vi "DAQ Performance Test.vi"() -> ()   [LabVIEW 2021]
uses:
  ChannelCommon/typedef/Benchmark Stats.ctl
  ChannelCommon/typedef/Direction.ctl
  CIF_Iceoryx_Fifo_DAQ.lvclass
  D:/dev/Packages/CIF_Channels_Core/src/CIFChannels/CIFChannels.lvclass
  Iceorxy Utilities/Typedef/DAQ FIFO Config.ctl
  ChannelCommon/typedef/Datatype Waveform.ctl
  <vilib>/Platform/TimedLoop/XDataNode/timing_clust.ctl
  <vilib>/Platform/TimedLoop/XDataNode/nitl_modes.ctl
  <vilib>/Platform/TimedLoop/XDataNode/wakeup.ctl
  ChannelCommon/typedef/TimeStamps.ctl
  CIFChannels/CIFChannels.lvclass/CIFChannels.ctl
  <vilib>/CIF Foundation/CIF Utilities/Statistics/I64/Stats_I64_CIF_U.lvclass/Stats_I64_CIF_U.ctl
  <vilib>/CIF Foundation/CIF Utilities/Statistics/I64/Get Stats.vi
  <vilib>/Platform/TimedLoop/XDataNode/XDataNode.xnode
  <vilib>/Platform/TimedLoop/XDataNode/XDNodeRunTimeDep.lvlib
  ChannelCommon/ChannelCommon.lvlib
  CIFChannels/CIFChannels.lvclass
  Iceorxy Utilities/Iceoryx Channel Utilities.lvlib
panel:
  out "timed out? 2":bool
  out "Channel W (us)":T1
  out "Flatten (us)":T1
  in  "stop":bool
  out "Unflatten (us)":T1
  out "Channel R (us)":T1
  out "timed out?":bool
  out "avg channel":dbl
  out "max channel":dbl
  out "pass":bool
  out "error out":errorcluster
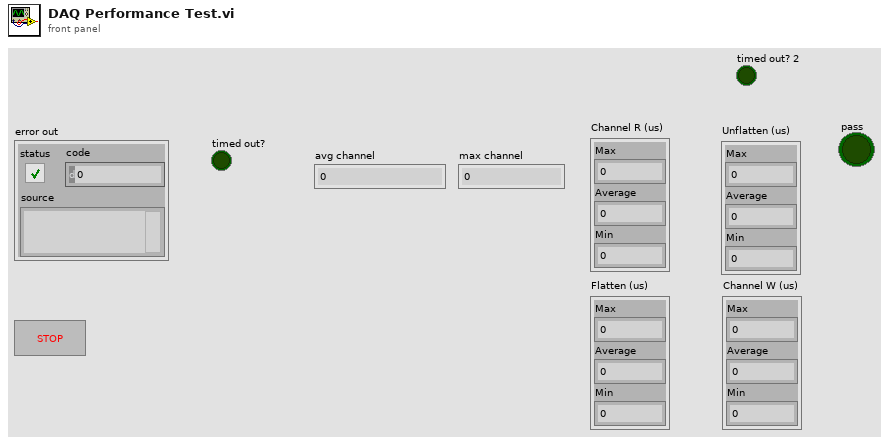
[diagram p1: front panel]
types:
  T1 = typedef "ChannelCommon.lvlib/Benchmark Stats.ctl" = cluster{"Max":i64, "Average":dbl, "Min":i64}
  T2 = typedef "Iceoryx Channel Utilities.lvlib/DAQ FIFO Config.ctl" = cluster{"Max Samples":u64, "Max Channels":u64, "FIFO Flags":cluster{"Backpressure":bool}, "Best Effort Subscribers":u32, "Backpressure Subscribers":u32}
  T3 = typedef "ChannelCommon.lvlib/Direction.ctl" = enum8{"Publisher", "Subscriber"}
  T4 = typedef "ChannelCommon.lvlib/Datatype Waveform.ctl" = cluster{"Measurement":dbl[], "dT":dbl, "Timestamp":i64}
  T5 = typedef "ChannelCommon.lvlib/TimeStamps.ctl" = cluster{"ClockID":u8, "T0":i64, "T_Out":i64}
  T6 = typedef "XDNodeRunTimeDep.lvlib/timing_clust.ctl" = cluster{"Expected End [f-1]":u64, "Actual End [f-1]":u64, "Finished Late? [f-1]":bool, "Expected End [i-1]":u64, "Actual End [i-1]":u64, "Finished Late? [i-1]":bool, "Expected Start [i]":u64, "Actual Start [i]":u64, "Expected Start [f]":u64, "Actual Start [f]":u64, "Source Name":string, "Structure Name":string, "Period":i64, "Deadline":i64, "Offset":i64, "Start":i64, "Priority":i32, "Timeout":i32, "Mode":T7, "Wakeup Reason":T8, "Error":errorcluster, "Source Type":string, "Secondary Source Type":string, "Global End Time":u64, "Global Start Time":u64, "Frame Duration":u64, "Iteration Duration":u64, "Assigned CPU":i32, "I/O Scan Engine Mode":u32}
  T7 = typedef "XDNodeRunTimeDep.lvlib/nitl_modes.ctl" = enum32{"No Change", "Process missed periods, maintain original phase", "Discard missed periods, maintain original phase", "Process missed periods, ignore original phase", "Discard missed periods, ignore original phase"}
  T8 = typedef "XDNodeRunTimeDep.lvlib/wakeup.ctl" = enum32{"Normal", "Aborted", "Asynchronous wakeup", "Timing source error", "Timed loop error", "Timeout"}
  T9 = typedef "ChannelCommon.lvlib/New FIFO Instance Response.ctl" = cluster{"Publisher":string, "Custom Data":u8[]}
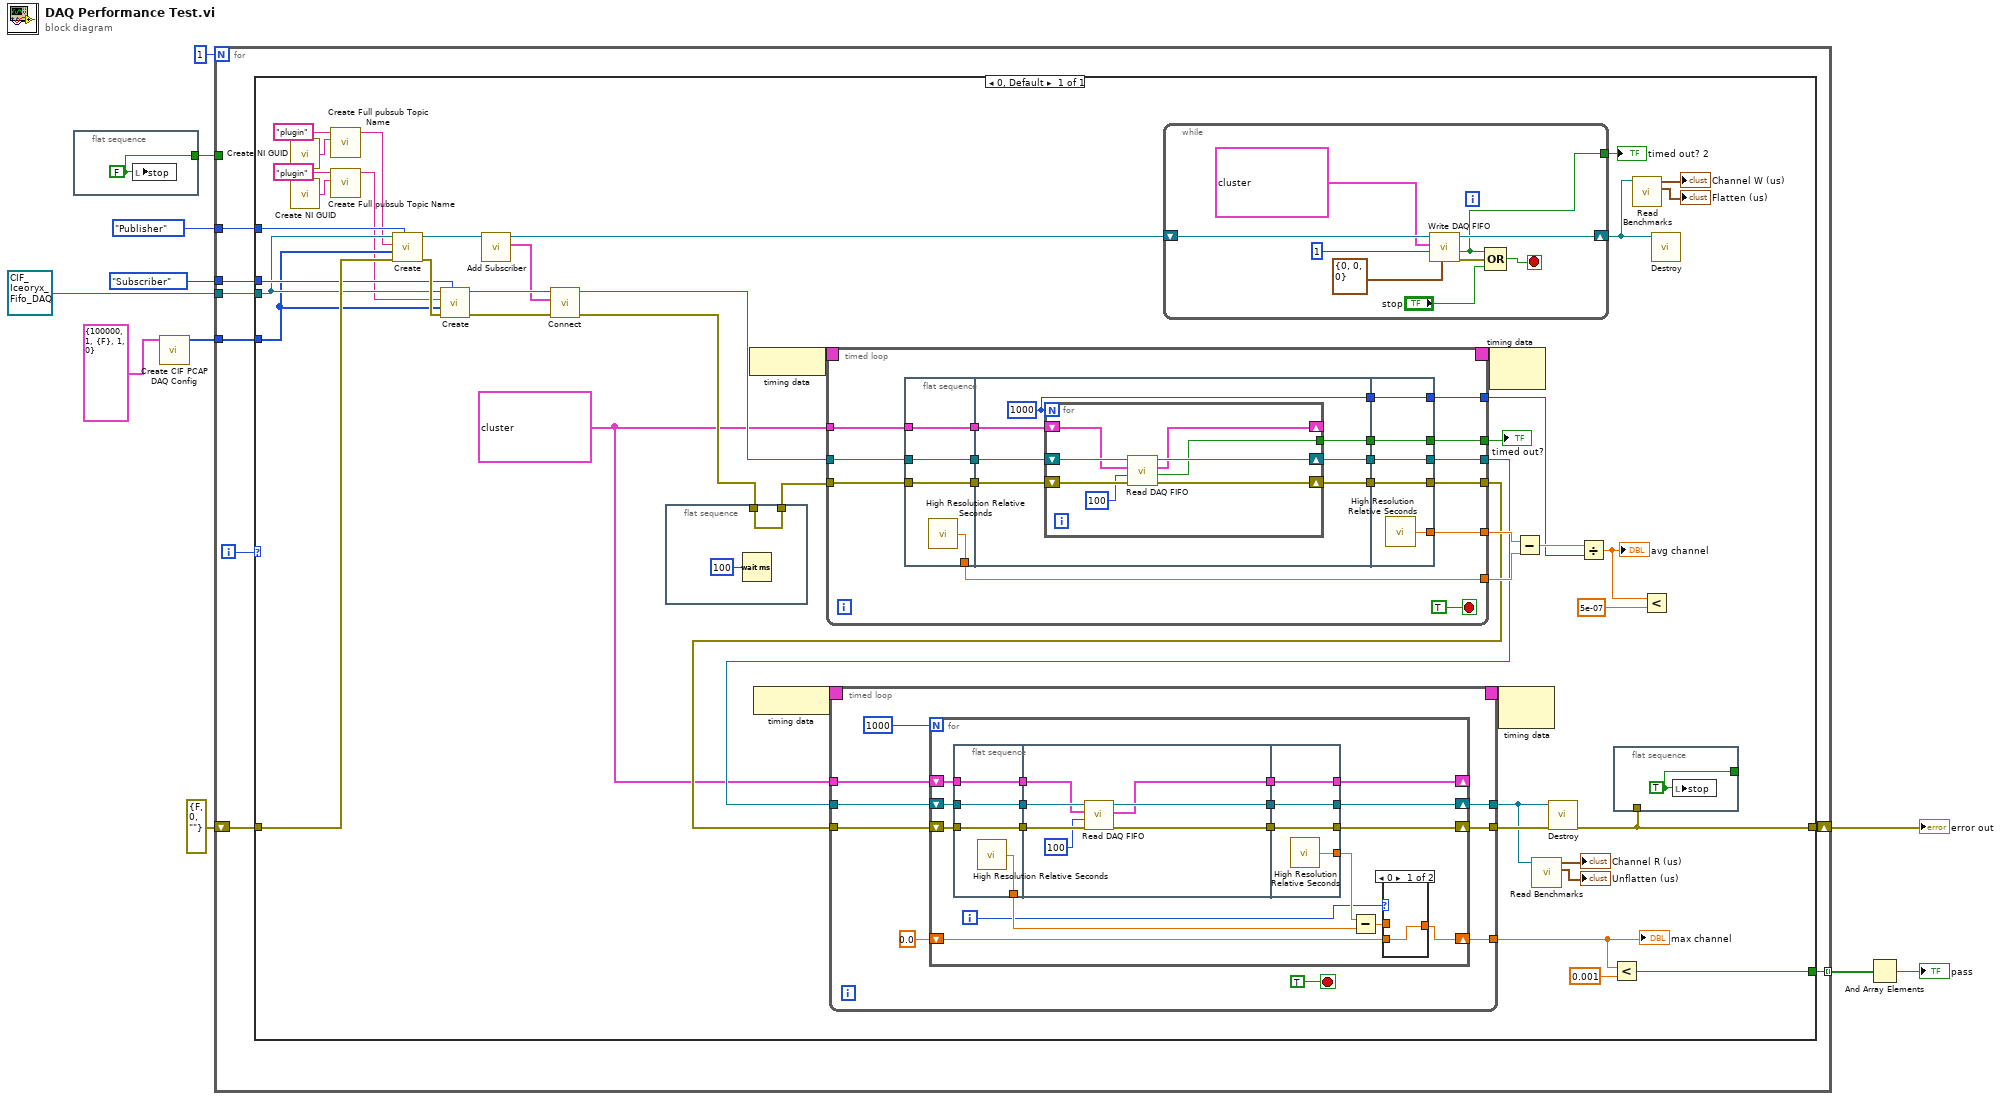
[diagram p0: block diagram]
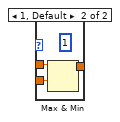
[diagram p2: hidden frame]
diagram:
  n1 = flat-sequence {
    tunnel: [w12] -> w3
    frame #0 {
      w12 = FALSE ("stop")
      n2 = local write "stop"(w12) -> ()
    }
  }
  n3 = call "Create CIF PCAP DAQ Config.vi"("DAQ FIFO Config"=T2 {"Max Samples"=100000, "Max Channels"=1, "FIFO Flags"={"Backpressure"=FALSE}, "Best Effort Subscribers"=1, "Backpressure Subscribers"=0}) -> ("Flattened FIFO Config"=w1:u8[])  [unwired: 10 in]
  n4 = for {
    N: 1 -> [_]
    tunnel: [w20] -> w9 mode=indexing
    shift-right: [w19] -> w11
    shift-left: errorcluster {"status"=FALSE, "code"=0, "source"=""} ("error out") -> [w17]
    tunnel: Direction."Publisher" ("Direction") -> [w16]
    tunnel: Direction."Subscriber" ("Direction") -> [w15]
    tunnel: refnum<class "CIF_Iceoryx_Fifo_DAQ.lvclass"> refnum ("CIF_CIPC_Fifo_U8.lvclass") -> [w14]
    tunnel: w1 -> [w13]
    tunnel: w3 -> [_]
    i -> [w18]
    n5 = case shown="0, Default" w18 {
      tunnel: [w52] -> w20
      tunnel: [w35] -> w19
      tunnel: w17 -> [w50]
      tunnel: w16 -> [w49]
      tunnel: w15 -> [w48]
      tunnel: w14 -> [w47]
      tunnel: w13 -> [w44]
      frame 0, Default {
        w28 = T4[] [{"Measurement"=array[100000 elements], "dT"=3.0, "Timestamp"=121}] ("Data In")
        n6 = call <vilib>:"Create NI GUID.vi"() -> ("NI GUID"=w30:string)
        n7 = call <vilib>:"Create NI GUID.vi"() -> ("NI GUID"=w31:string)
        n8 = call "Create Full pubsub Topic Name.vi"("Topic"=w30, "Plugin name"="plugin") -> ("Full Topic"=w27:string)  [unwired: 8 in, 1 out]
        n9 = call "Create Full pubsub Topic Name.vi"("Topic"=w31, "Plugin name"="plugin") -> ("Full Topic"=w26:string)  [unwired: 8 in, 1 out]
        n10 = call-dynamic "Create.vi"("Direction"=w49, "error in (no error)"=w50, "Custom Config Data"=w44, "Name"=w27, "CIFFIFO in"=w47) -> ("error out"=w51:errorcluster, "CIFFIFO out"=w34:refnum<class "CIF_Iceoryx_Fifo_DAQ.lvclass">)  [unwired: 5 in]
        n11 = call-dynamic "Create.vi"("Direction"=w48, "error in (no error)"=w51, "Custom Config Data"=w44, "Name"=w26, "CIFFIFO in"=w47) -> ("error out"=w45:errorcluster, "CIFFIFO out"=w46:refnum<class "CIF_Iceoryx_Fifo_DAQ.lvclass">)  [unwired: 5 in]
        n12 = call-dynamic "Add Subscriber.vi"("CIF_CIPC_Chn in"=w34) -> ("New FIFO Instance"=w33:T9, "CIF_CIPC_Chn out"=w23:refnum<class "CIF_Iceoryx_Fifo_DAQ.lvclass">)  [unwired: 8 in, 1 out]
        n13 = call-dynamic "Connect.vi"("error in (no error)"=w45, "Connection"=w33, "CIF_Iceoryx_PCAP"=w46) -> ("error out"=w41:errorcluster, "CIF_Iceoryx_PCAP"=w43:refnum<class "CIF_Iceoryx_Fifo_DAQ.lvclass">)  [unwired: 7 in]
        n14 = flat-sequence {
          tunnel: w41 -> [w69]
          tunnel: [w69] -> w40
          frame #0 {
            n15 = Wait (ms)(milliseconds to wait=u32 100) -> ()  [unwired: 1 out]
          }
        }
        n16 = node-c288() -> (w66:T6)
        n17 = node-c288() -> (w64:T6)
        n18 = timed-loop {
          timing: w66 -> [_]
          timing-out: [_] -> w65
          tunnel: w43 -> [w145]
          tunnel: w40 -> [w144]
          tunnel: [w140] -> w58
          tunnel: [w138] -> w57
          tunnel: [w136] -> w62
          tunnel: [w135] -> w61
          tunnel: [w134] -> w59
          tunnel: [w132] -> w39
          tunnel: w28 -> [w129]
          stop <- TRUE stop-if-true
          n19 = flat-sequence {
            tunnel: w144 -> [w148]
            tunnel: w145 -> [w149]
            tunnel: [w149] -> w142
            tunnel: [w148] -> w141
            tunnel: [w147] -> w135
            tunnel: [w146] -> w130
            tunnel: w129 -> [w146]
            tunnel: w142 -> [w156]
            tunnel: w141 -> [w155]
            tunnel: [w154] -> w139
            tunnel: [w153] -> w137
            tunnel: [w152] -> w133
            tunnel: [w151] -> w131
            tunnel: w130 -> [w150]
            tunnel: [w169] -> w140
            tunnel: w139 -> [w169]
            tunnel: [w168] -> w138
            tunnel: w137 -> [w168]
            tunnel: [w167] -> w136
            tunnel: [w166] -> w134
            tunnel: w133 -> [w166]
            tunnel: [w165] -> w132
            tunnel: w131 -> [w165]
            frame #0 {
              n20 = call <vilib>:"High Resolution Relative Seconds.vi"() -> ("relative seconds"=w147:dbl)
            }
            frame #1 {
              w152 = 1000
              n21 = for {
                N: w152 -> [_]
                shift-right: [w161] -> w154
                shift-left: w156 -> [w164]
                shift-right: [w162] -> w153
                shift-left: w155 -> [w163]
                tunnel: [w159] -> w151
                shift-right: [w157] -> _
                shift-left: w150 -> [w158]
                n22 = call-dynamic "Read DAQ FIFO.vi"("error in (no error)"=w163, "Timeout (ms)"=100, "Data In"=w158, "CIFFIFO in"=w164) -> ("error out"=w162:errorcluster, "timed out?"=w159:bool, "Data Out"=w157:T4[], "CIFFIFO out"=w161:refnum<class "CIF_Iceoryx_Fifo_DAQ.lvclass">)  [unwired: 3 in, 1 out]
              }
            }
            frame #2 {
              n23 = call <vilib>:"High Resolution Relative Seconds.vi"() -> ("relative seconds"=w167:dbl)
            }
          }
        }
        "timed out?" <- w39
        n24 = timed-loop {
          timing: w64 -> [_]
          timing-out: [_] -> w63
          tunnel: w58 -> [w87]
          tunnel: w57 -> [w86]
          tunnel: [w84] -> w38
          tunnel: [w83] -> w42
          tunnel: [w80] -> w54
          tunnel: w28 -> [w79]
          stop <- TRUE stop-if-true
          n25 = for {
            N: 1000 -> [_]
            shift-right: [w100] -> w84
            shift-left: w87 -> [w102]
            shift-right: [w99] -> w83
            shift-left: w86 -> [w101]
            shift-right: [w94] -> w80
            shift-left: 0.0 -> [w95]
            shift-right: [w89] -> _
            shift-left: w79 -> [w90]
            i -> [w93]
            n26 = flat-sequence {
              tunnel: w101 -> [w112]
              tunnel: w102 -> [w113]
              tunnel: [w113] -> w105
              tunnel: [w112] -> w104
              tunnel: [w111] -> w97
              tunnel: [w110] -> w91
              tunnel: w90 -> [w110]
              tunnel: w105 -> [w120]
              tunnel: w104 -> [w119]
              tunnel: [w117] -> w103
              tunnel: [w118] -> w92
              tunnel: w91 -> [w115]
              tunnel: [w114] -> w88
              tunnel: [w124] -> w100
              tunnel: w103 -> [w124]
              tunnel: [w123] -> w99
              tunnel: [w122] -> w98
              tunnel: w92 -> [w123]
              tunnel: [w121] -> w89
              tunnel: w88 -> [w121]
              frame #0 {
                n27 = call <vilib>:"High Resolution Relative Seconds.vi"() -> ("relative seconds"=w111:dbl)
              }
              frame #1 {
                n28 = call-dynamic "Read DAQ FIFO.vi"("error in (no error)"=w119, "Timeout (ms)"=100, "Data In"=w115, "CIFFIFO in"=w120) -> ("error out"=w118:errorcluster, "Data Out"=w114:T4[], "CIFFIFO out"=w117:refnum<class "CIF_Iceoryx_Fifo_DAQ.lvclass">)  [unwired: 3 in, 2 out]
              }
              frame #2 {
                n29 = call <vilib>:"High Resolution Relative Seconds.vi"() -> ("relative seconds"=w122:dbl)
              }
            }
            n30 = Subtract(x=w98, y=w97) -> (x-y=w96:dbl)
            n31 = case shown="0" w93 {
              tunnel: w96 -> [_ w109]
              tunnel: w95 -> [w106 w108]
              tunnel: [w106 w107] -> w94
              frame 0 {
              }
              frame 1, Default {
                (unwired) u32 1 ("milliseconds to wait")
                n32 = Max & Min(x=w109, y=w108) -> (max(x,y)=w107:dbl)  [unwired: 1 out]
              }
            }
          }
        }
        "max channel" <- w54
        n33 = while {
          shift-right: [w76] -> w24
          shift-left: w23 -> [w78]
          tunnel: [w70] -> w22
          stop <- w75 stop-if-true
          n34 = call-dynamic "Write DAQ FIFO.vi"("FIFO Timestamps"=T5 {"ClockID"=0, "T0"=0, "T_Out"=0}, "Timeout (ms)"=1, "Data In"=T4[] [{"Measurement"=array[100000 elements], "dT"=3.0, "Timestamp"=121}], "CIFFIFO in"=w78) -> ("error out"=w71:errorcluster, "timed out?"=w70:bool, "CIFFIFO out"=w76:refnum<class "CIF_Iceoryx_Fifo_DAQ.lvclass">)  [unwired: 4 in, 1 out]
          n35 = Compound Arithmetic op=OR(w70, w71, "stop") -> (w75:bool)
        }
        "timed out? 2" <- w22
        n36 = node-c288(w65) -> ()  [unwired: 1 out]
        n37 = node-c288(w63) -> ()  [unwired: 1 out]
        n38 = Subtract(x=w62, y=w61) -> (x-y=w60:dbl)
        n39 = call "Read Benchmarks.vi"("CIFChannels in"=w38) -> ("Flatten (us)"=→"Unflatten (us)":T1, "Channel R/W (us)"=→"Channel R (us)":T1)  [unwired: 9 in]
        n40 = call-dynamic "Destroy.vi"("error in (no error)"=w42, "Icoryx_PCAP in"=w38) -> ("error out"=w35:errorcluster)  [unwired: 8 in, 1 out]
        n41 = Divide(x=w60, y=w59) -> (x/y=w56:dbl)
        "avg channel" <- w56
        n42 = Less?(x=w54, y=0.001) -> (x < y?=w52:bool)
        n43 = flat-sequence {
          tunnel: [w67] -> _
          tunnel: w35 -> [_]
          frame #0 {
            w67 = TRUE ("stop")
            n44 = local write "stop"(w67) -> ()
          }
        }
        n45 = call "Read Benchmarks.vi"("CIFChannels in"=w24) -> ("Flatten (us)"=→"Flatten (us)":T1, "Channel R/W (us)"=→"Channel W (us)":T1)  [unwired: 9 in]
        n46 = Less?(x=w56, y=5e-07) -> ()  [unwired: 1 out]
        n47 = call-dynamic "Destroy.vi"("Icoryx_PCAP in"=w24) -> ()  [unwired: 9 in, 2 out]
      }
    }
  }
  "error out" <- w11
  n48 = And Array Elements(Boolean array=w9) -> (logical AND=→"pass":bool)
